vi "Limit AO DC.vi"(8 "error in (no error)":errorcluster, 11 "Instrument.DAQ":refnum<class "Instrument.DAQ.lvclass">) -> (0 "error out":errorcluster, 3 "Instrument.DAQ out":refnum<class "Instrument.DAQ.lvclass">)   [LabVIEW 2019, in "Instrument.Lockin.lvlib" / "Instrument.DAQ.lvclass"]
uses:
  Instrument.DAQ.lvclass
  Instrument.DAQ.lvclass/Instrument.DAQ.ctl
  5eead935-39ba-4ca3-950f-9e334bf8d01b.vi
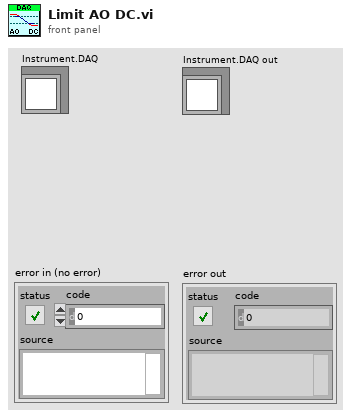
[diagram p1: front panel]
types:
  T1 = typedef "Instrument.Lockin.lvlib/Instrument.DAQ.lvclass/AO.Channel--Cluster--Array.ctl" = T2[]
  T2 = typedef "Instrument.Lockin.lvlib/Instrument.DAQ.lvclass/AO.Channel--Cluster.ctl" = cluster{"Enable?":bool, "Channel":i32, "Amplitude":dbl, "Offset":dbl, "Frequency":dbl, "Phase":dbl, "Function":T3, "Sweeping?":bool, "Limit AC":bool, "Limit DC?":bool, "Function Option":bool}
  T3 = typedef "Instrument.Lockin.lvlib/Instrument.DAQ.lvclass/AO.Channel.Function--Enum.ctl" = enum16{"sine", "triangle", "square"}
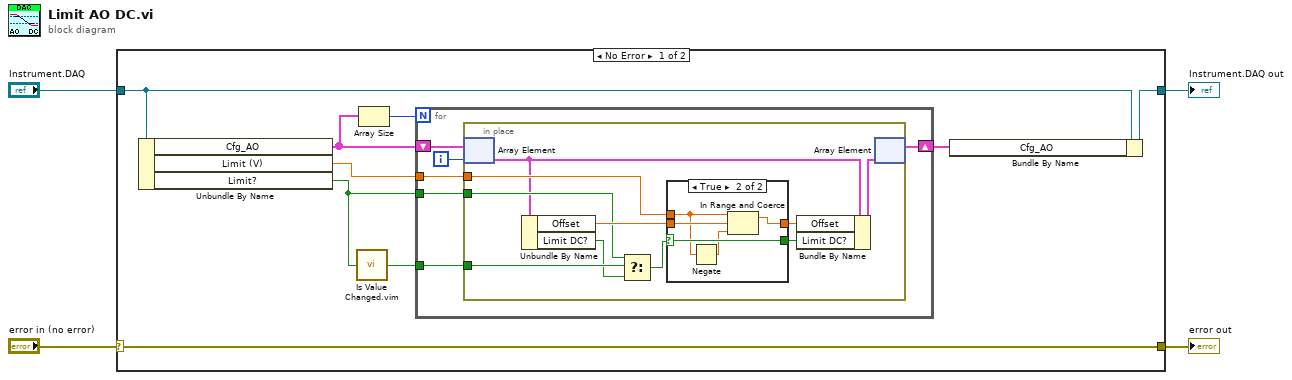
[diagram p0: block diagram]
diagram:
  n1 = case shown="No Error" "error in (no error)" {
    selector: "error in (no error)" -> [w11 w38]
    tunnel: [w13 w37] -> w4
    tunnel: "Instrument.DAQ" -> [w12 w37]
    tunnel: [w11 w38] -> w2
    frame No Error {
      n2 = Unbundle By Name(w12) -> ("Cfg_AO"=w6:T1, "Limit (V)"=w10:dbl, "Limit?"=w9:bool)
      n3 = call "Is Value Changed.vim"("value"=w9) -> ("changed or first call?"=w8:bool)
      n4 = Array Size(array=w6) -> (size(s)=w7:i32)
      n5 = for {
        N: w7 -> [_]
        tunnel: w10 -> [w19]
        tunnel: w8 -> [w18]
        tunnel: w9 -> [w17]
        shift-right: [w14] -> w5
        shift-left: w6 -> [w16]
        i -> [w15]
        n6 = in-place {
          in-place-border: w19 -> [w26]
          in-place-border: w18 -> [w25]
          in-place-border: w17 -> [w24]
          n7 = in-place-array #1(w16, w15) -> (w21:T2)
          n8 = Unbundle By Name(w21) -> ("Offset"=w29:dbl, "Limit DC?"=w23:bool)
          n9 = Select(t=w24, s=w25, f=w23) -> (s? t:f=w22:bool)
          n10 = case shown="True" w22 {
            selector: w22 -> [w30 w34]
            tunnel: w29 -> [w31 w36]
            tunnel: w26 -> [_ w33]
            tunnel: [w31 w35] -> w28
            tunnel: [w30 w34] -> w27
            frame False {
            }
            frame True {
              n11 = Negate(x=w33) -> (-x=w32:dbl)
              n12 = In Range and Coerce(upper limit=w33, x=w36, lower limit=w32) -> (coerced(x)=w35:dbl)  [unwired: 1 out]
            }
          }
          n13 = Bundle By Name(cluster=w21, "Offset"=w28, "Limit DC?"=w27) -> (w20:T2)
          n14 = in-place-array #1(w20) -> (w14:T1)  [unwired: 1 out]
        }
      }
      n15 = Bundle By Name(cluster=w12, "Cfg_AO"=w5) -> (w13:refnum<class "Instrument.DAQ.lvclass">)
    }
    frame Error {
    }
  }
  "Instrument.DAQ out" <- w4
  "error out" <- w2
